vi "create stream from rid.vi"(7 "fallback avro file (user documents\\nominal_fallback_files)":path, 10 "Dataset RID":string, 11 "API Key":string) -> (0 "error out":errorcluster, 3 "stream session":refnum<data-value>)   [LabVIEW 2020, in "nominal core steps.lvlib"]
doc: "Create a reference to a stream to a provided dataset RID without obtaining the dataset reference first."
uses:
  nominal core steps.lvlib
  stream session.ctl
  <vilib>/Nominal/Nominal IO Client/submodules/nominal-streaming-labview-ffi/lv_src/Stream/Stream.lvclass
  channel uid.ctl
  <vilib>/Nominal/Nominal IO Client/submodules/nominal-streaming-labview-ffi/lv_src/Channel/Channel.lvclass
  <vilib>/Utility/sysdir.llb/System Directory Type.ctl
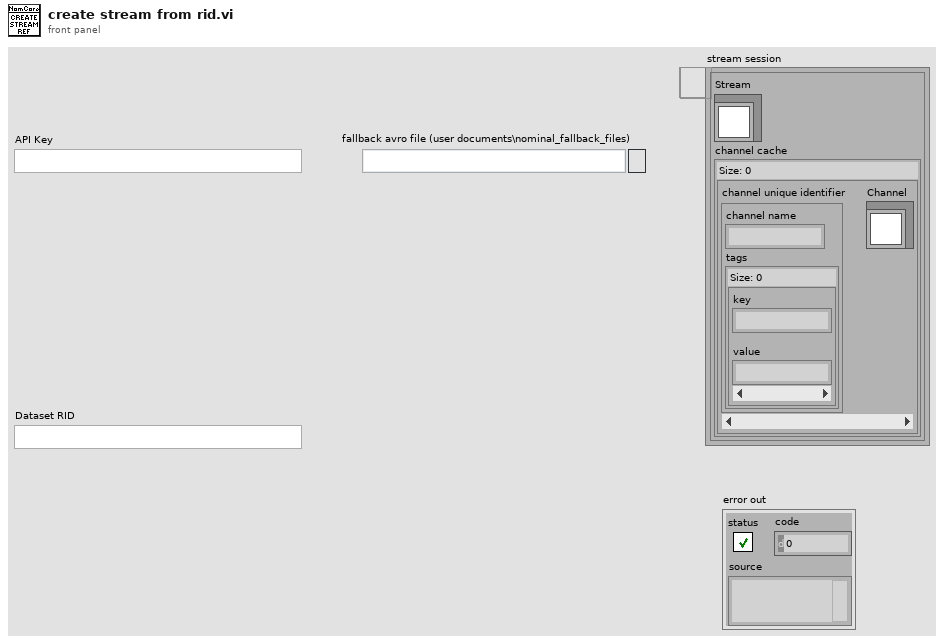
[diagram p1: front panel]
types:
  T1 = typedef "System Directory Type.ctl" = i32
  T2 = typedef "nominal core steps.lvlib/stream session.ctl" = cluster{"Stream":refnum<class "Stream.lvclass">, "channel cache":map{T3, refnum<class "Channel.lvclass">}}
  T3 = typedef "nominal core steps.lvlib/channel uid.ctl" = cluster{"channel name":string, "tags":map{string, string}}
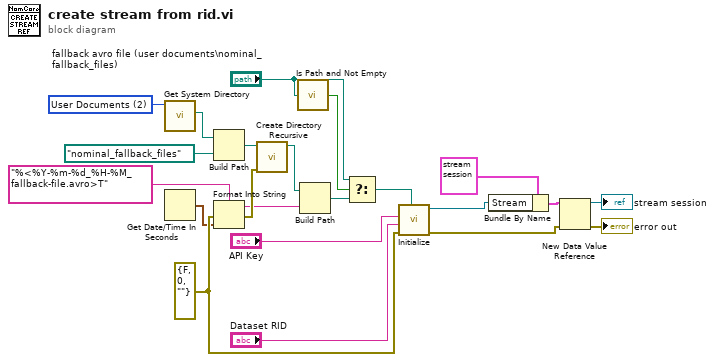
[diagram p0: block diagram]
diagram:
  w8 = T1 2 items=["User Home"=0, "User Desktop"=1, "User Documents"=2, "User Application Data"=3, "User Preferences"=4, "User Temporary"=5, "Public Documents"=6, "Public Application Data"=7, "Public Preferences"=8, "Public Cache"=13, "System Core Libraries"=9, "System Installed Libraries"=10, "Application Files"=11, "Boot Volume Root"=12] ("system directory type")
  w15 = errorcluster {"status"=FALSE, "code"=0, "source"=""} ("error in (no error)")
  n1 = call <vilib>:"Get System Directory.vi"("system directory type"=w8) -> ("system directory"=w7:path)  [unwired: 10 in]
  n2 = Get Date/Time In Seconds() -> (seconds since 1Jan1904=w5:timestamp)
  n3 = Build Path(base path=w7, name or relative path=path "nominal_fallback_files") -> (appended path=w9:path)
  n4 = Format Into String(format string="%<%Y-%m-%d_%H-%M_fallback-file.avro>T", error in=w15, w5) -> (resulting string=w6:string, error out=w11:errorcluster)  [unwired: 1 in]
  n5 = call <vilib>:"Create Directory Recursive.vi"("error in (no error)"=w11, "directory"=w9) -> ("directory copy"=w10:path)  [unwired: 3 in, 2 out]
  n6 = call <vilib>:"Is Path and Not Empty.vi"("path"="fallback avro file (user documents\\nominal_fallback_files)") -> ("Is Path and Not Empty?"=w12:bool)  [unwired: 4 in]
  n7 = Build Path(base path=w10, name or relative path=w6) -> (appended path=w13:path)
  n8 = Select(t="fallback avro file (user documents\\nominal_fallback_files)", s=w12, f=w13) -> (s? t:f=w14:path)
  n9 = call <vilib>:"Initialize.vi"("Fallback File Path"=w14, "error in (no error)"=w15, "Dataset RID"="Dataset RID", "Token"="API Key") -> ("error out"=w22:errorcluster, "Nominal Streaming out"=w19:refnum<class "Stream.lvclass">)  [unwired: 6 in]
  n10 = Bundle By Name(cluster=T2 {"Stream"=refnum, "channel cache"={}} ("stream session"), "Stream"=w19) -> (w18:T2)
  n11 = New Data Value Reference(data value=w18, error in=w22) -> (data value reference=→"stream session":refnum<data-value>, error out=→"error out":errorcluster)
